vi "Own20261012_GetConnectorInfo.vi"() -> ()   [LabVIEW 2024]
uses:
  <vilib>/Utility/miscctls.llb/LVRectTypeDef.ctl
panel:
  out "control_ids":refnum<vi>[](array[refnum])
  out "terminal_bounds":T1[](array[typedef])
  out "terminal_count":u32
  out "pattern":u32
  out "error out":errorcluster caption="错误输出"
  in  "target_path":path
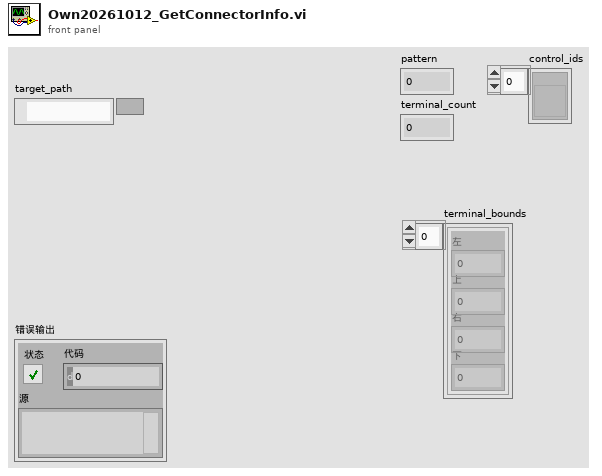
[diagram p1: front panel]
types:
  T1 = typedef "LVRectTypeDef.ctl" = cluster{"Left":i16, "Top":i16, "Right":i16, "Bottom":i16}
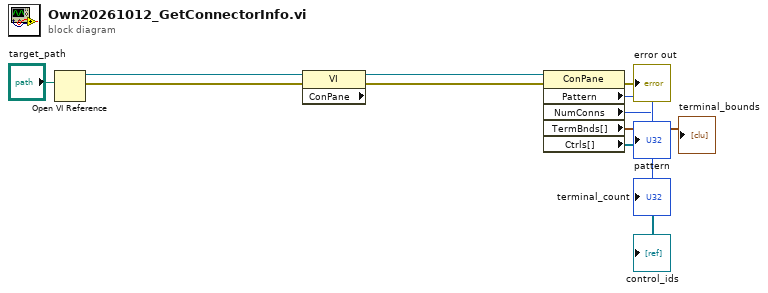
[diagram p0: block diagram]
diagram:
  n1 = Open VI Reference ("打开VI引用")(vi path="target_path") -> (vi reference=w9:refnum<vi>, error out=w8:errorcluster)  [unwired: 5 in]
  n2 = property on="属性节点" class="VI"(reference=w9, error in=w8) -> (error out=w6:errorcluster, "ConPane"=w7:refnum<vi>)  [unwired: 1 out]
  n3 = property on="属性节点" class="ConPane"(reference=w7, error in=w6) -> (error out=→"error out":errorcluster, "Pattern"=→"pattern":u32, "NumConns"=→"terminal_count":u32, "TermBnds[]"=→"terminal_bounds":T1[], "Ctrls[]"=→"control_ids":refnum<vi>[])  [unwired: 1 out]
